vi "Write Sequence.vi"(8 "error in (no error)":errorcluster, 10 "Sequence File":T1, 11 "Sequence Executor in":refnum<class "Sequence Executor.lvclass">) -> (0 "error out":errorcluster, 3 "Sequence Executor out":refnum<class "Sequence Executor.lvclass">)   [LabVIEW 2026, in "Sequence Executor.lvclass"]
doc: "Writes one field of this class's private data. Generated by lvai_create_accessors from the class private data control."
uses:
  Sequence Executor.lvclass
  Typedefs/Sequence File.ctl
  Typedefs/Step Config.ctl
  Typedefs/Channel Value.ctl
  Typedefs/Condition.ctl
  Sequence Executor.lvclass/Sequence Executor.ctl
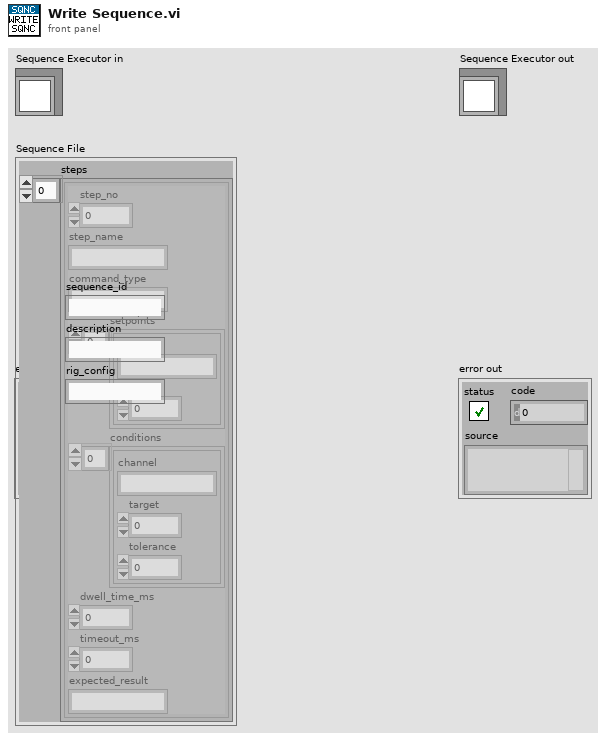
[diagram p1: front panel]
types:
  T1 = typedef "Sequence File.ctl" = cluster{"sequence_id":string, "description":string, "rig_config":string, "steps":T2[]}
  T2 = typedef "Step Config.ctl" = cluster{"step_no":i32, "step_name":string, "command_type":string, "setpoints":T3[], "conditions":T4[], "dwell_time_ms":i32, "timeout_ms":i32, "expected_result":string}
  T3 = typedef "Channel Value.ctl" = cluster{"channel":string, "value":dbl}
  T4 = typedef "Condition.ctl" = cluster{"channel":string, "target":dbl, "tolerance":dbl}
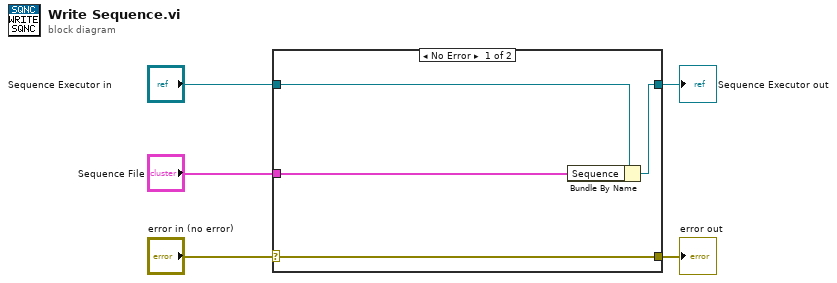
[diagram p0: block diagram]
diagram:
  n1 = case shown="No Error" "error in (no error)" {
    selector: "error in (no error)" -> [w9 w10]
    tunnel: [w9 w10] -> w4
    tunnel: [w7 w11] -> w2
    tunnel: "Sequence Executor in" -> [w8 w11]
    tunnel: "Sequence File" -> [w6 _]
    frame No Error {
      n2 = Bundle By Name(cluster=w8, "Sequence"=w6) -> (w7:refnum<class "Sequence Executor.lvclass">)
    }
    frame Error {
    }
  }
  "error out" <- w4
  "Sequence Executor out" <- w2
